vi "GV_TC9_Mo.vi"() -> ()   [LabVIEW 2025]
panel:
  out "TC_Monitor_TC9":dbl
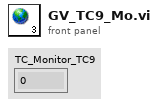
[diagram p1: front panel]
diagram:
